vi "Transport_Send_Event.vi"(8 "error in (no error)":errorcluster={"status"=FALSE, "code"=0, "source"="\"\""}, 10 "transport ref":string, 11 "EventRecord":string) -> (0 "error out":errorcluster={"status"=FALSE, "code"=0, "source"="\"\""}, 2 "status ok":bool, 3 "Delivery status":string)   [LabVIEW 2026]
doc: "INTENT: Publish event/status to Host. LOGIC: Serialize event with monotonically increasing event sequence; send on event channel."
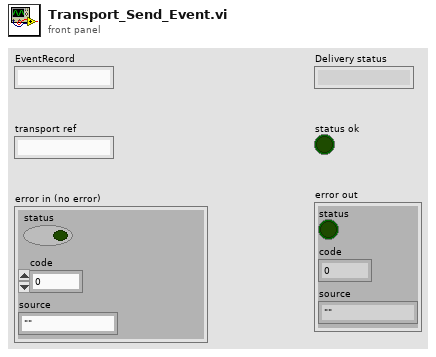
[diagram p1: front panel]
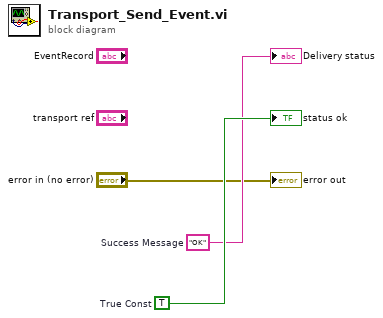
[diagram p0: block diagram]
diagram:
  w3 = TRUE  # True Const
  w2 = "OK"  # Success Message
  "Delivery status" <- w2
  "status ok" <- w3
  "error out" <- "error in (no error)"
